vi "SMC Checksum.vi"(10 "Pad":bool=TRUE, 11 "String in":string) -> (2 "Checksum String":string, 3 "result string":string)   [LabVIEW 2026, in "Protections.lvlib" / "SMC Protection.lvclass"]
uses:
  SMC Protection.lvclass
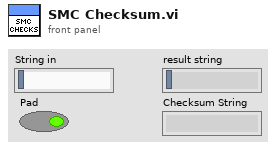
[diagram p1: front panel]
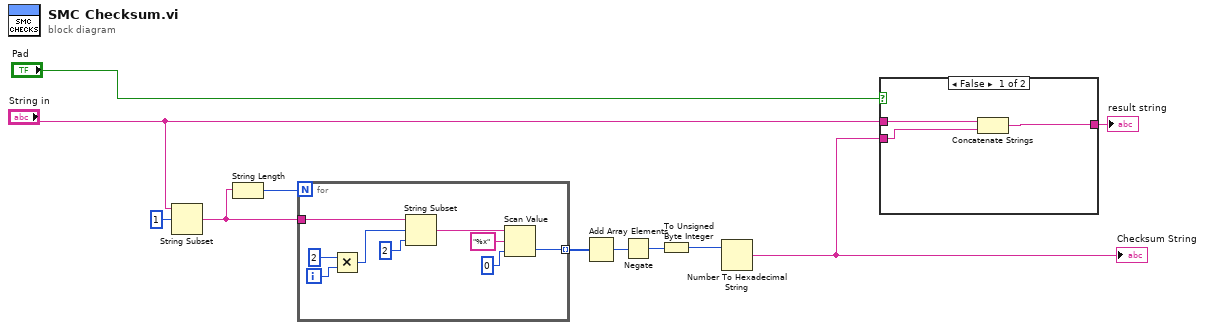
[diagram p0: block diagram]
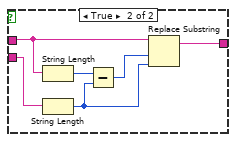
[diagram p2: hidden frame]
diagram:
  n1 = String Subset(string="String in", offset (0)=1) -> (substring=w6:string)  [unwired: 1 in]
  n2 = String Length(string=w6) -> (length=w7:i32)
  n3 = for {
    N: w7 -> [_]
    tunnel: w6 -> [w18]
    tunnel: [w12] -> w5 mode=indexing
    i -> [w20]
    n4 = Multiply(x=2, y=w20) -> (x*y=w17:i32)
    n5 = String Subset(string=w18, offset (0)=w17, length (rest)=2 ("x")) -> (substring=w15:string)
    n6 = Scan Value(string=w15, format string="%x", default (0 dbl)=0 ("x")) -> (value=w12:i32)  [unwired: 1 out]
  }
  n7 = Add Array Elements(numeric array=w5) -> (sum=w4:i32)
  n8 = Negate(x=w4) -> (-x=w3:i32)
  n9 = To Unsigned Byte Integer(number=w3) -> (unsigned 8bit integer=w2:u8)
  n10 = Number To Hexadecimal String(2:w2) -> (0:w1:string)  [unwired: 1 in]
  "Checksum String" <- w1
  n11 = case shown="False" "Pad" {
    tunnel: "String in" -> [w23 w28]
    tunnel: [w22 w29] -> w10
    tunnel: w1 -> [w21 w24]
    frame False {
      n12 = Concatenate Strings(w23, w21) -> (w22:string)
    }
    frame True {
      n13 = String Length(string=w28) -> (length=w27:i32)
      n14 = String Length(string=w24) -> (length=w26:i32)
      n15 = Subtract(x=w27, y=w26) -> (x-y=w25:i32)
      n16 = Replace Substring(2:w26, 3:w25, 5:w28) -> (1:w29:string)  [unwired: 1 in, 1 out]
    }
  }
  "result string" <- w10
